vi "VIH HelpGen - Get Control Terminal Image.vi"(8 "error in":errorcluster, 11 "Ctl Refnum":refnum<vi>) -> (0 "error out":errorcluster, 1 "Indicator":bool, 2 "Ctrl Term Icon":T1, 3 "dup Ctl Refnum":refnum<vi>, 4 "Data Type":variant)   [LabVIEW 2014]
doc: "::: VI Helpeks :::\nCopyright (c) 2000-2026 Konstantin Shifershteyn. All rights reserved."
uses:
  <vilib>/picture/picture.llb/imagedata.ctl
  <vilib>/Utility/miscctls.llb/LVPositionTypeDef.ctl
panel:
  # "VI Helpeks\nCopyright (c) 2012-2026 Konstantin Shifershteyn"
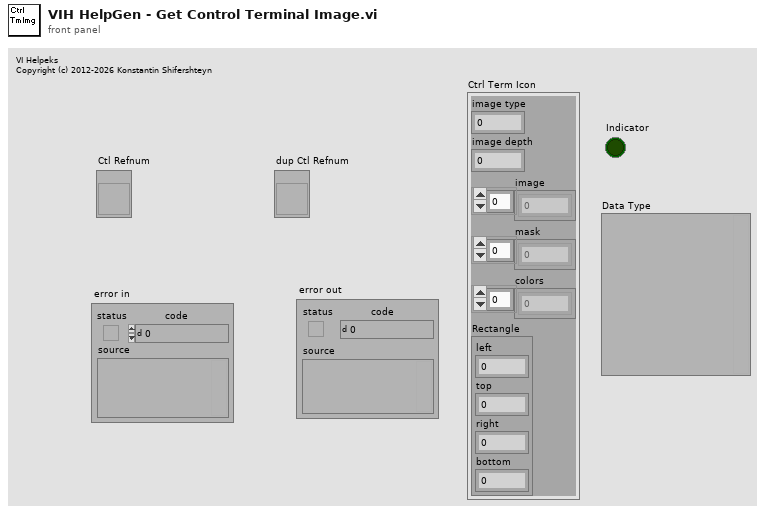
[diagram p1: front panel]
types:
  T1 = typedef "imagedata.ctl" = cluster{"image type":i32, "image depth":i32, "image":u8[], "mask":u8[], "colors":u32[], "Rectangle":cluster{"left":i16, "top":i16, "right":i16, "bottom":i16}}
  T2 = typedef "LVPositionTypeDef.ctl" = cluster{"Left":i32, "Top":i32}
  T3 = cluster{"left":i16, "top":i16, "right":i16, "bottom":i16}
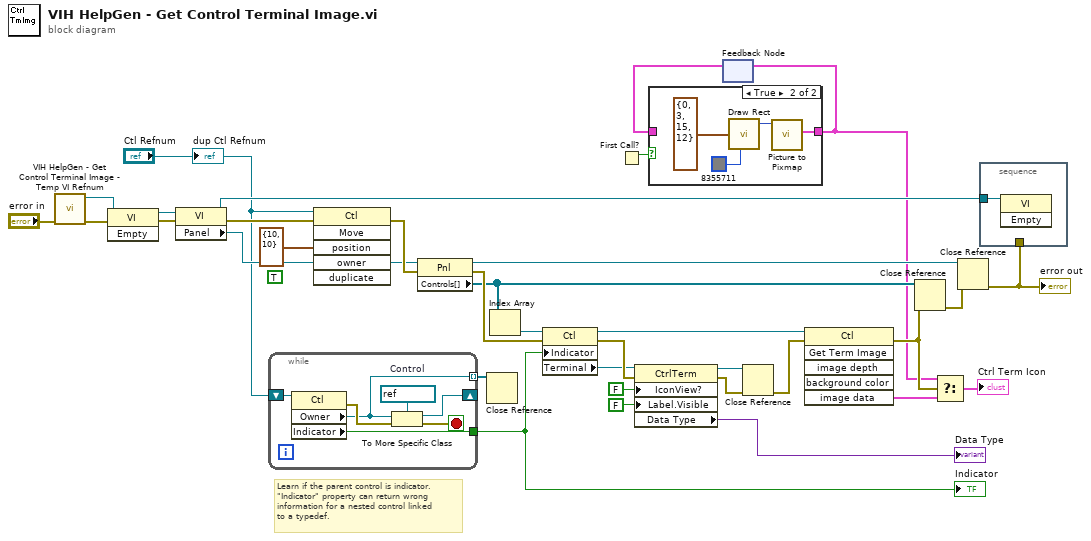
[diagram p0: block diagram]
diagram:
  (unwired) TRUE
  # "Learn if the parent control is indicator.\n\"Indicator\" property can return wrong\ninformation for a nested control linked\nto a typedef."
  n1 = call "VIH HelpGen - Get Control Terminal Image - Temp VI Refnum.vi"("error in"="error in") -> ("error out"=w7:errorcluster, "VI Refnum"=w33:refnum<vi>)  [unwired: 9 in]
  n2 = invoke class="VI" method="Empty"(reference=w33, error in=w7) -> (reference out=w32:refnum<vi>, error out=w31:errorcluster)  [unwired: 1 in, 1 out]
  n3 = property class="VI"(reference=w32, error in=w31) -> (reference out=w18:refnum<vi>, error out=w30:errorcluster, "Panel"=w28:refnum<vi>)
  n4 = while {
    tunnel: [w38] -> w9
    shift-right: [w37] -> _
    shift-left: "Ctl Refnum" -> [w39]
    tunnel: [w35] -> w10 mode=indexing
    stop <- w36 stop-if-true
    w40 = refnum<vi> refnum  # Control
    n5 = property class="Ctl"(reference=w39) -> (error out=w41:errorcluster, "Owner"=w35:refnum<vi>, "Indicator"=w38:bool)  [unwired: 1 in, 1 out]
    n6 = To More Specific Class(target class=w40, reference=w35, error in=w41) -> (specific class reference=w37:refnum<vi>, error out=w36:errorcluster)
  }
  "Indicator" <- w9
  n7 = invoke class="Ctl" method="Move"(reference="Ctl Refnum", error in=w30, "position"=T2 {"Left"=10, "Top"=10}, "owner"=w28) -> (error out=w29:errorcluster)  [unwired: 2 in, 5 out]
  n8 = property class="Pnl"(reference=w28, error in=w29) -> (reference out=w17:refnum<vi>, error out=w20:errorcluster, "Controls[]"=w19:refnum<vi>[])
  n9 = Close Reference(reference=w10) -> ()  [unwired: 1 in, 1 out]
  n10 = Index Array(array=w19) -> (element=w13:refnum<vi>)  [unwired: 1 in]
  n11 = property class="Ctl"(reference=w13, error in=w20, "Indicator"=w9) -> (reference out=w21:refnum<vi>, error out=w25:errorcluster, "Terminal"=w12:refnum<vi>)
  n12 = First Call?() -> (First Call?: T/F=w6:bool)
  n13 = property class="CtrlTerm"(reference=w12, error in=w25, "IconView?"=FALSE ("Icon View?"), "Label.Visible"=FALSE) -> (reference out=w24:refnum<vi>, error out=w26:errorcluster, "Data Type"=→"Data Type":variant)
  n14 = feedback #1() -> (w5:T1)  [unwired: 1 in]
  n15 = case shown="True" w6 {
    tunnel: [w42 w43] -> w1
    tunnel: w5 -> [w42 _]
    frame False {
    }
    frame True {
      n16 = call <vilib>:"Draw Rect.vi"("rect"=T3 {"left"=0, "top"=3, "right"=15, "bottom"=12}, "color(black)"=u32 8355711) -> ("new picture"=w44:picture)  [unwired: 7 in]
      n17 = call <vilib>:"Picture to Pixmap.vi"("picture"=w44) -> ("image data"=w43:T1)  [unwired: 9 in, 1 out]
    }
  }
  n18 = feedback-in #1(w1) -> ()
  n19 = Close Reference(reference=w24, error in (no error)=w26) -> (error out=w27:errorcluster)
  n20 = invoke class="Ctl" method="Get Term Image"(reference=w21, error in=w27) -> (error out=w3:errorcluster, "image data"=w4:T1)  [unwired: 4 in, 4 out]
  n21 = Close Reference(reference=w19, error in (no error)=w3) -> (error out=w16:errorcluster)
  n22 = Select(t=w1, s=w3, f=w4) -> (s? t:f=→"Ctrl Term Icon":T1)
  n23 = Close Reference(reference=w17, error in (no error)=w16) -> (error out=w15:errorcluster)
  "error out" <- w15
  n24 = stacked-sequence {
    tunnel: w18 -> [w47]
    tunnel: w15 -> [_]
    frame #0 {
      n25 = invoke class="VI" method="Empty"(reference=w47) -> ()  [unwired: 2 in, 3 out]
    }
  }
  "dup Ctl Refnum" <- "Ctl Refnum"
